vi "Read INI File.vi"(8 "error in":errorcluster, 11 "Peer Review in":refnum<class "Peer Review.lvclass">) -> (0 "error out":errorcluster, 3 "Peer Review out":refnum<class "Peer Review.lvclass">)   [LabVIEW 2020, in "Peer Review.lvclass"]
uses:
  Peer Review.lvclass
  Peer Review.lvclass/Peer Review.ctl
  <vilib>/Utility/config.llb/Read Key (Path).vi
  <vilib>/Utility/config.llb/Read Key (Boolean).vi
  <vilib>/Utility/config.llb/Read Key (String).vi
  <vilib>/Utility/config.llb/NI_LVConfig.lvlib
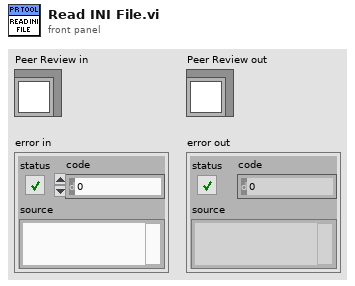
[diagram p1: front panel]
types:
  T1 = typedef "NI_LVConfig.lvlib/Config Data RefNum.ctl" = refnum<k1>
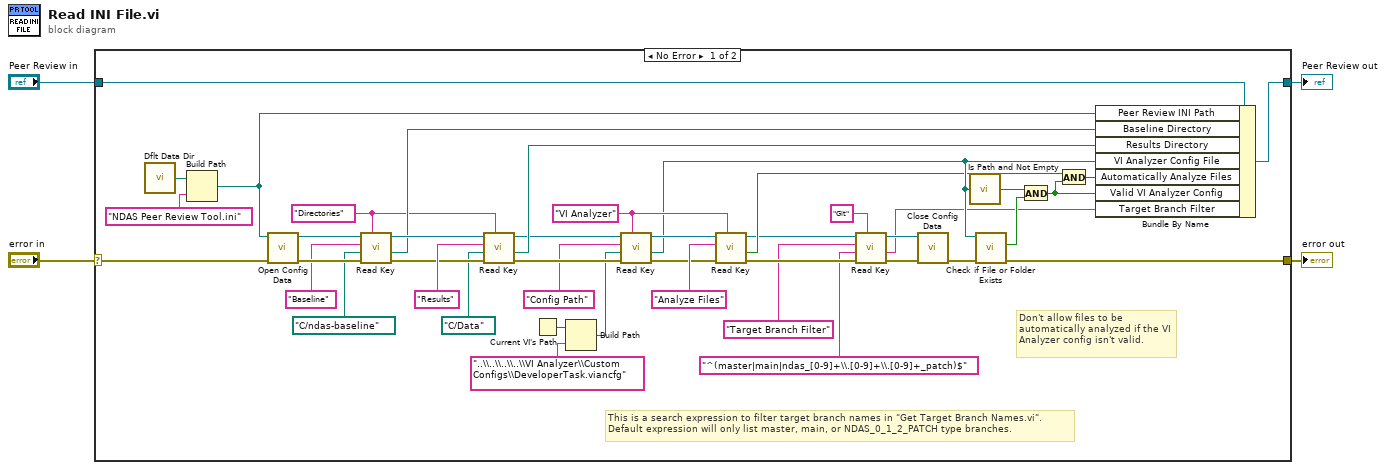
[diagram p0: block diagram]
diagram:
  n1 = case shown="No Error" "error in" {
    selector: "error in" -> [w40 w49]
    tunnel: [w21 w49] -> w3
    tunnel: "Peer Review in" -> [w23 w48]
    tunnel: [w36 w48] -> w1
    frame No Error {
      w24 = "VI Analyzer" ("section")
      w28 = "Directories" ("section")
      # "This is a search expression to filter target branch names in \"Get Target Branch Names.vi\".\nDefault expression will only list master, main, or NDAS_0_1_2_PATCH type branches."
      # "Don't allow files to be automatically analyzed if the VI Analyzer config isn't valid."
      n2 = call <vilib>:"Dflt Data Dir.vi"() -> ("App:Default Data Directory"=w13:path)
      n3 = Build Path(base path=w13, name or relative path="NDAS Peer Review Tool.ini") -> (appended path=w19:path)
      n4 = call <vilib>:"Open Config Data.vi"("error in (no error)"=w40, "configuration file path"=w19) -> ("error out"=w46:errorcluster, "refnum"=w45:T1)  [unwired: 7 in, 1 out]
      n5 = call-poly <vilib>:"Read Key.vi"("section"=w28, "error in (no error)"=w46, "default value"=path "C:/ndas-baseline" ("Baseline Directory"), "key"="Baseline" ("section"), "refnum"=w45) -> ("error out"=w41:errorcluster, "value"=w37:path, "refnum out"=w44:T1)  [unwired: 3 in, 1 out]
      n6 = call-poly <vilib>:"Read Key.vi"("section"=w28, "error in (no error)"=w41, "default value"=path "C:/Data" ("Results Directory"), "key"="Results" ("section"), "refnum"=w44) -> ("error out"=w31:errorcluster, "value"=w35:path, "refnum out"=w32:T1)  [unwired: 3 in, 1 out]
      n7 = Current VI's Path() -> (path=w33:path)
      n8 = Build Path(base path=w33, name or relative path="..\\..\\..\\..\\VI Analyzer\\Custom Configs\\DeveloperTask.viancfg") -> (appended path=w25:path)
      n9 = call-poly <vilib>:"Read Key.vi"("section"=w24, "error in (no error)"=w31, "default value"=w25, "key"="Config Path" ("section"), "refnum"=w32) -> ("error out"=w29:errorcluster, "value"=w20:path, "refnum out"=w30:T1)  [unwired: 3 in, 1 out]
      n10 = call-poly <vilib>:"Read Key.vi"("section"=w24, "error in (no error)"=w29, "key"="Analyze Files", "refnum"=w30) -> ("error out"=w9:errorcluster, "value"=w16:bool, "refnum out"=w12:T1)  [unwired: 4 in, 1 out]
      n11 = call-poly <vilib>:"Read Key.vi"("section"="Git", "error in (no error)"=w9, "default value"="^(master|main|ndas_[0-9]+\\.[0-9]+\\.[0-9]+_patch)$", "key"="Target Branch Filter", "refnum"=w12) -> ("error out"=w10:errorcluster, "value"=w5:string, "refnum out"=w11:T1)  [unwired: 3 in, 1 out]
      n12 = call <vilib>:"Close Config Data.vi"("error in (no error)"=w10, "refnum"=w11) -> ("error out"=w22:errorcluster)  [unwired: 8 in, 1 out]
      n13 = call <vilib>:"Is Path and Not Empty.vi"("path"=w20) -> ("Is Path and Not Empty?"=w18:bool)  [unwired: 4 in]
      n14 = call <vilib>:"Check if File or Folder Exists.vi"("error in (no error)"=w22, "path"=w20) -> ("error out"=w21:errorcluster, "file or folder exists?"=w17:bool)  [unwired: 7 in, 1 out]
      n15 = And(x=w18, y=w17) -> (x .and. y?=w15:bool)
      n16 = And(x=w16, y=w15) -> (x .and. y?=w14:bool)
      n17 = Bundle By Name(cluster=w23, "Peer Review INI Path"=w19, "Baseline Directory"=w37, "Results Directory"=w35, "VI Analyzer Config File"=w20, "Automatically Analyze Files"=w14, "Valid VI Analyzer Config"=w15, "Target Branch Filter"=w5) -> (w36:refnum<class "Peer Review.lvclass">)
    }
    frame Error {
    }
  }
  "error out" <- w3
  "Peer Review out" <- w1
